vi "Review Branch.vi"(8 "error in":errorcluster, 11 "Peer Review in":refnum<class "Peer Review.lvclass">) -> (0 "error out":errorcluster, 3 "Peer Review out":refnum<class "Peer Review.lvclass">)   [LabVIEW 2020, in "Peer Review.lvclass"]
uses:
  Peer Review.lvclass
  Peer Review.lvclass/Peer Review.ctl
  <vilib>/Utility/cursorutil.llb/Set Cursor (Icon Pict).vi
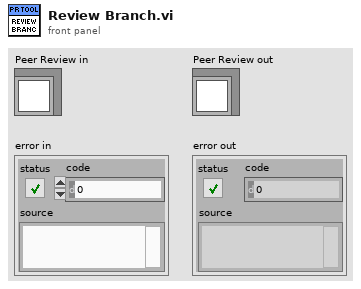
[diagram p1: front panel]
types:
  T1 = enum32{"Commit History", "File List", "Git Log", "Description", "Image"}
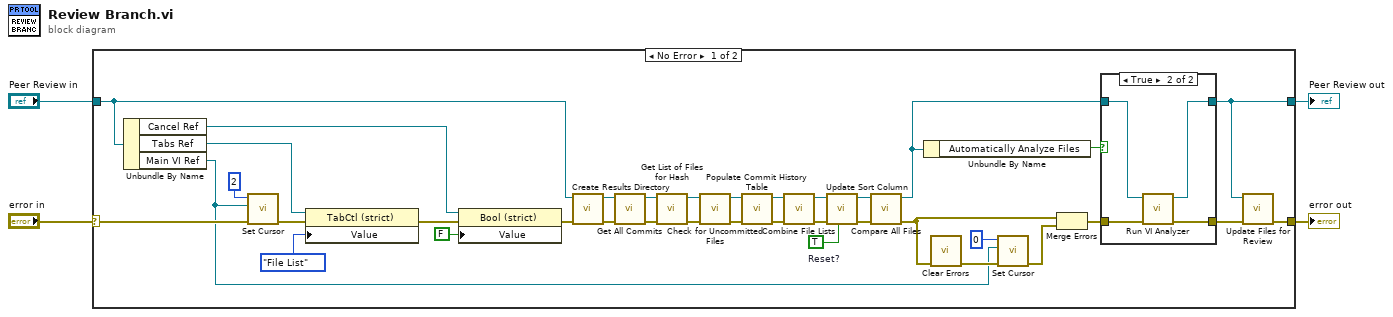
[diagram p0: block diagram]
diagram:
  n1 = case shown="No Error" "error in" {
    selector: "error in" -> [w22 w48]
    tunnel: [w7 w48] -> w4
    tunnel: "Peer Review in" -> [w19 w47]
    tunnel: [w6 w47] -> w1
    frame No Error {
      w33 = TRUE  # Reset?
      n2 = Unbundle By Name(w19) -> ("Cancel Ref"=w11:refnum<vi>, "Tabs Ref"=w34:refnum<vi>, "Main VI Ref"=w15:refnum<vi>)
      n3 = call-poly <vilib>:"Set Cursor.vi"("error in (no error)"=w22, "VI reference (current VI)"=w15, "icon"=u16 2) -> ("error out"=w21:errorcluster)  [unwired: 7 in, 1 out]
      n4 = property on="Property Node" class="TabCtl (strict)"(reference=w34, error in=w21, "Value"=T1."File List") -> (error out=w8:errorcluster)  [unwired: 1 out]
      n5 = property on="Property Node" class="Bool (strict)"(reference=w11, error in=w8, "Value"=FALSE) -> (error out=w9:errorcluster)  [unwired: 1 out]
      n6 = call "Create Results Directory.vi"("error in"=w9, "Peer Review in"=w19) -> ("error out"=w40:errorcluster, "Peer Review out"=w37:refnum<class "Peer Review.lvclass">)  [unwired: 8 in]
      n7 = call "Get All Commits.vi"("error in"=w40, "Peer Review in"=w37) -> ("error out"=w36:errorcluster, "Peer Review out"=w35:refnum<class "Peer Review.lvclass">)  [unwired: 8 in]
      n8 = call "Get List of Files for Hash.vi"("error in"=w36, "Peer Review in"=w35) -> ("error out"=w28:errorcluster, "Peer Review out"=w29:refnum<class "Peer Review.lvclass">)  [unwired: 8 in]
      n9 = call "Check for Uncommitted Files.vi"("error in"=w28, "Peer Review in"=w29) -> ("error out"=w27:errorcluster, "Peer Review out"=w26:refnum<class "Peer Review.lvclass">)  [unwired: 8 in]
      n10 = call "Populate Commit History Table.vi"("error in"=w27, "Peer Review in"=w26) -> ("error out"=w31:errorcluster, "Peer Review out"=w30:refnum<class "Peer Review.lvclass">)  [unwired: 8 in]
      n11 = call "Combine File Lists.vi"("error in"=w31, "Peer Review in"=w30) -> ("error out"=w38:errorcluster, "Peer Review out"=w39:refnum<class "Peer Review.lvclass">)  [unwired: 8 in]
      n12 = call "Update Sort Column.vi"("Reset?"=w33, "error in"=w38, "Peer Review in"=w39) -> ("error out"=w24:errorcluster, "Peer Review out"=w25:refnum<class "Peer Review.lvclass">)  [unwired: 7 in]
      n13 = call "Compare All Files.vi"("error in"=w24, "Peer Review in"=w25) -> ("error out"=w13:errorcluster, "Peer Review out"=w17:refnum<class "Peer Review.lvclass">)  [unwired: 8 in]
      n14 = Unbundle By Name(w17) -> ("Automatically Analyze Files"=w18:bool)
      n15 = call <vilib>:"Clear Errors.vi"("error in (no error)"=w13) -> ("error out"=w16:errorcluster)  [unwired: 5 in, 1 out]
      n16 = call-poly <vilib>:"Set Cursor.vi"("error in (no error)"=w16, "VI reference (current VI)"=w15, "icon"=u16 0) -> ("error out"=w14:errorcluster)  [unwired: 7 in, 1 out]
      n17 = Merge Errors(w13, w14) -> (w12:errorcluster)
      n18 = case shown="True" w18 {
        tunnel: w17 -> [w42 w46]
        tunnel: [w42 w45] -> w6
        tunnel: w12 -> [w41 w44]
        tunnel: [w41 w43] -> w5
        frame False {
        }
        frame True {
          n19 = call "Run VI Analyzer.vi"("error in"=w44, "Peer Review in"=w46) -> ("error out"=w43:errorcluster, "Peer Review out"=w45:refnum<class "Peer Review.lvclass">)  [unwired: 8 in]
        }
      }
      n20 = call "Update Files for Review.vi"("error in"=w5, "Peer Review"=w6) -> ("error out"=w7:errorcluster)  [unwired: 9 in]
    }
    frame Error {
    }
  }
  "error out" <- w4
  "Peer Review out" <- w1
